vi "P1.vi"() -> ()   [LabVIEW 2025]
uses:
  <vilib>/MakerHub/LINX/Public/Peripherals/Analog/Analog Read 1 Chan.vi
  <vilib>/MakerHub/LINX/Public/Peripherals/Digital/Digital Write 1 Chan.vi
  <vilib>/MakerHub/LINX/Public/Peripherals/Digital/Digital Read 1 Chan.vi
  <vilib>/MakerHub/LINX/Public/Peripherals/Analog/Analog Read N Chans.vi
  <vilib>/MakerHub/LINX/Public/Peripherals/Digital/Digital Write N Chans.vi
  <vilib>/MakerHub/LINX/Public/Peripherals/Digital/Digital Read N Chans.vi
  <vilib>/MakerHub/LINX/Private/Local IO/LinxAnalogRead.vi
  <vilib>/MakerHub/LINX/Public/Utilities/Check Channel.vi
  <vilib>/MakerHub/LINX/Private/Local IO/LinxDigitalWrite.vi
  <vilib>/MakerHub/LINX/Private/Local IO/LinxDigitalRead.vi
  <vilib>/MakerHub/LINX/Public/Utilities/Open Serial.vi
  <vilib>/MakerHub/LINX/Private/Utilties/Generate Error.vi
  <vilib>/MakerHub/LINX/LMH-LINX.lvlib
panel:
  in  "Serial Port":refnum<visa-resource-name>="N/A"
  out "NIVEL":string
  out "TANQUE":dbl(slide) scale=0.0..10.0
  out "<10":bool
  out ">100":bool
  out "°K":dbl(slide) scale=0.0..500.0
  out "°F":dbl(slide) scale=0.0..500.0
  out "°C":dbl(slide) scale=0.0..500.0
  out "RAIZ CUADRADA":dbl
  out "DIVISION":dbl
  out "MULTIPLICACION":dbl
  out "SUMA":dbl
  in  "N2":dbl
  in  "N1":dbl
  out "PANTALLA":string
  in  "TEXTO":string
  out "Led puerta":bool
  in  "Puerta":bool
  in  "stop":bool
  in  "Control °C":dbl(slide) scale=0.0..200.0
  out "°C":dbl(slide) scale=0.0..200.0
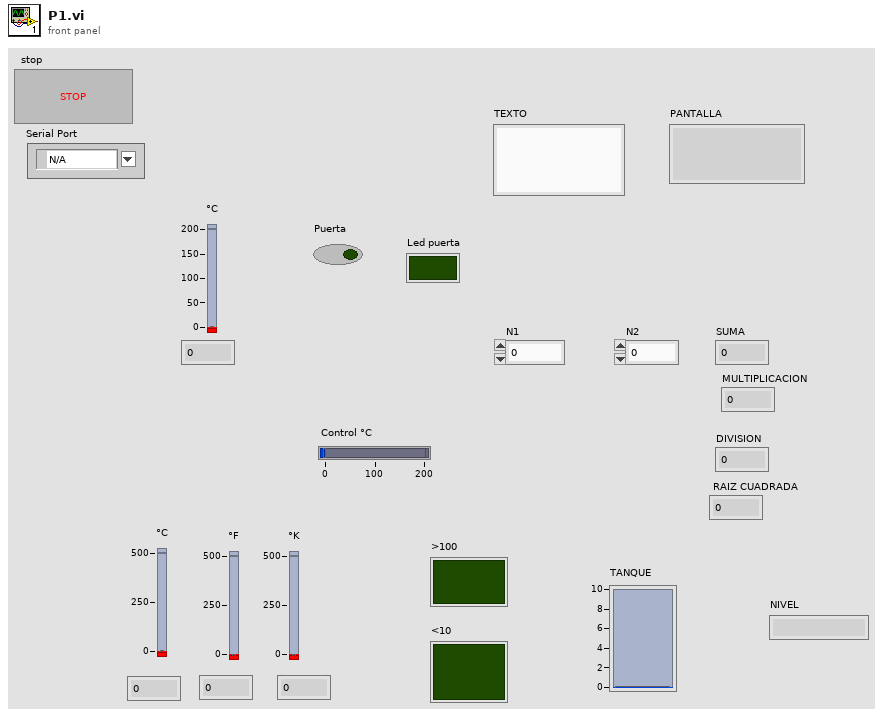
[diagram p1: front panel]
types:
  T1 = typedef "LMH-LINX.lvlib/LINX Ref.ctl" = cluster{"IO":T2, "Interface":T3, "LINX Device Config":T4}
  T2 = typedef "LMH-LINX.lvlib/Platform.ctl" = enum16{"Remote", "Local"}
  T3 = typedef "LMH-LINX.lvlib/Interface.ctl" = enum16{"Serial", "TCP"}
  T4 = typedef "LMH-LINX.lvlib/Device.lvlib/LINX Device Config.ctl" = cluster{"Interface":T3, "COM Port":refnum<visa-resource-name>, "TCP Configuration":T5, "Device Family":u8, "Device ID":u8, "Device Name":string, "TCP Ref":refnum<k5>, "Channels":T6}
  T5 = typedef "LMH-LINX.lvlib/Device.lvlib/TCP Config.ctl" = cluster{"IP Address":string, "Port":u16}
  T6 = typedef "LMH-LINX.lvlib/Channels.ctl" = cluster{"DI":u8[], "DO":u8[], "AI":u8[], "AO":u8[], "PWM":u8[], "QE":u8[], "UART":u8[], "I2C 2":u8[], "SPI":u8[], "CAN":u8[], "Servo":u8[], "AI Ref (V)":dbl, "AI Resolution (Bits)":u8, "AO Ref (V)":dbl, "AO Resolution (Bits)":u8}
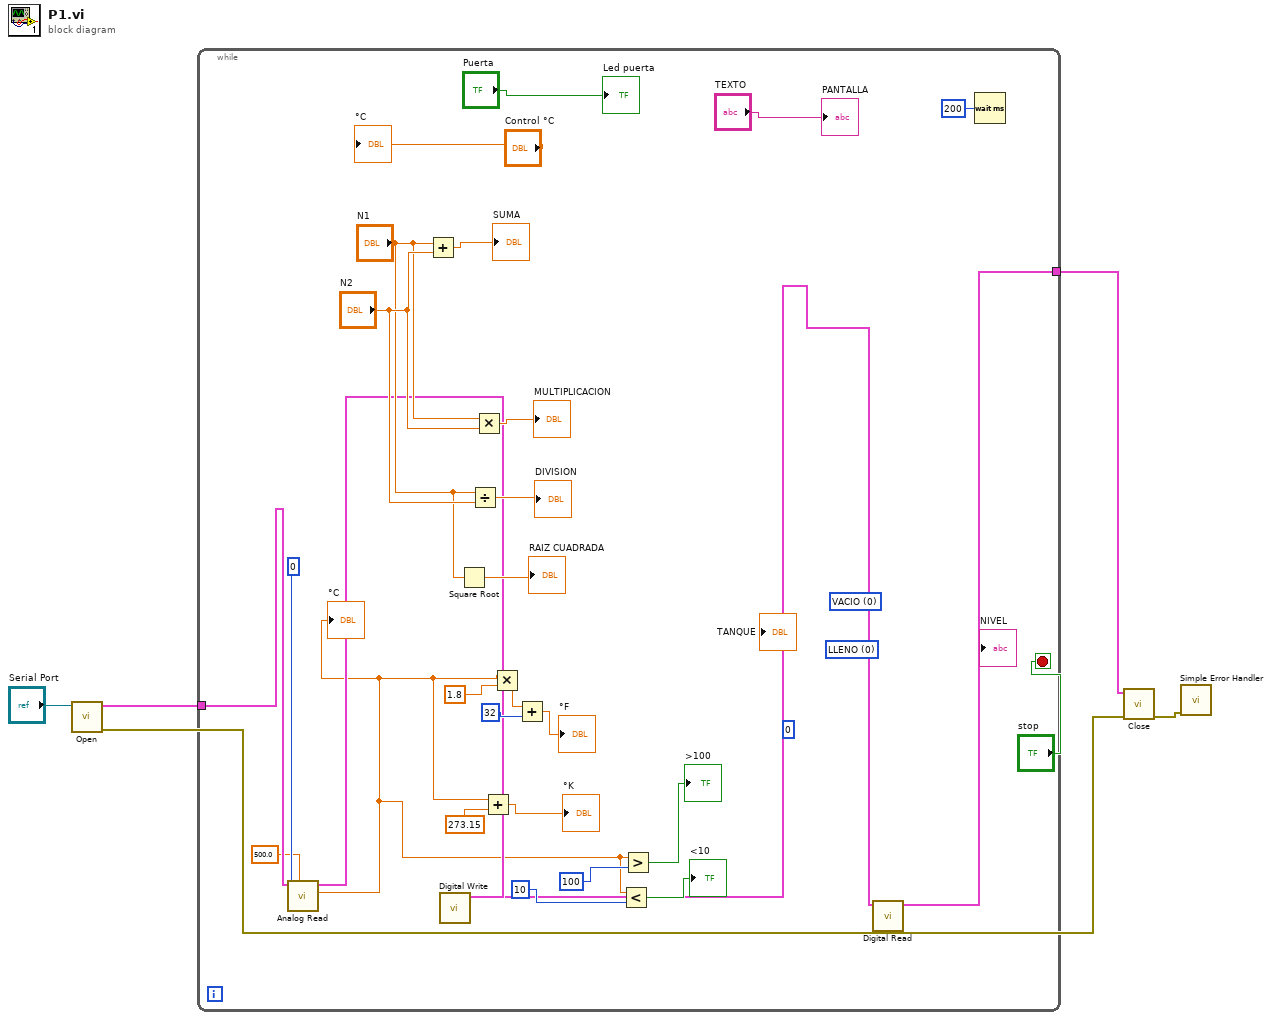
[diagram p0: block diagram]
diagram:
  n1 = call-poly <vilib>:"Open.vi"("Serial Port"="Serial Port") -> ("Error Out"=w2:errorcluster, "LINX Resource"=w5:T1)  [unwired: 8 in, 1 out]
  n2 = while {
    tunnel: w5 -> [w12]
    tunnel: [w9] -> w4
    stop <- "stop" stop-if-true
    (unwired) 0
    (unwired) u16 0 items=["LLENO"]
    (unwired) u16 0 items=["VACIO"]
    n3 = call-poly <vilib>:"Analog Read.vi"("Analog Ref Override (V)"=500.0, "Analog Channel"=u8 0, "LINX Resource"=w12) -> ("Voltage"=w7:dbl, "LINX Resource"=w11:T1)  [unwired: 5 in, 2 out]
    "°C" <- w7
    n4 = Add(x="N1", y="N2") -> (x+y=→"SUMA":dbl)
    n5 = call-poly <vilib>:"Digital Write.vi"("LINX Resource"=w11) -> ("LINX Resource"=w10:T1)  [unwired: 9 in, 1 out]
    n6 = Square Root(x="N1") -> (sqrt(x)=→"RAIZ CUADRADA":dbl)
    n7 = Divide(x="N1", y="N2") -> (x/y=→"DIVISION":dbl)
    n8 = Multiply(x="N1", y="N2") -> (x*y=→"MULTIPLICACION":dbl)
    n9 = Add(x=w7, y=273.15) -> (x+y=→"°K":dbl)
    n10 = Multiply(x=w7, y=1.8) -> (x*y=w21:dbl)
    n11 = Add(x=w21, y=32) -> (x+y=→"°F":dbl)
    n12 = Less?(x=w7, y=10) -> (x < y?=→"<10":bool)
    n13 = Greater?(x=w7, y=100) -> (0:→">100":bool)
    n14 = call-poly <vilib>:"Digital Read.vi"("LINX Resource"=w10) -> ("LINX Resource"=w9:T1)  [unwired: 8 in, 2 out]
    n15 = Wait (ms)(milliseconds to wait=u32 200) -> ()  [unwired: 1 out]
    "°C" <- "Control °C"
    "Led puerta" <- "Puerta"
    "PANTALLA" <- "TEXTO"
  }
  n16 = call <vilib>:"Close.vi"("Error In"=w2, "LINX Resource"=w4) -> ("Error Out"=w1:errorcluster)  [unwired: 9 in]
  n17 = call <vilib>:"Simple Error Handler.vi"("error in (no error)"=w1) -> ()  [unwired: 4 in, 5 out]
